vi "4Pi Interference Locator.vi"(7 "Calling VI Ref":refnum<vi>) -> ()   [LabVIEW 2021]
uses:
  <vilib>/vision/Image Controls.llb/IMAQ Image.ctl
  Hardware Configuration/Hardware Configuration Controls/Device Type.ctl
  Hardware Configuration/Hardware Configuration Controls/Device Function.ctl
  Device Library/Stages/Stages Controls/Stage Actions.ctl
  <vilib>/Utility/miscctls.llb/LVPointTypeDef.ctl
  4Pi Interference Locator Type Defs/4Pi IL Notifier Type.ctl
  4Pi Interference Locator Type Defs/4Pi IL Actions.ctl
  Device Manager/Common Device Queue/Common Device Controls/Common Device Actions.ctl
  Device Library/Cameras/Hamamatsu/Orca Flash/Orca Flash Controls/Orca Flash Actions.ctl
  Display Module/Display Module Custom Controls/ROI Descriptor.ctl
  Device Library/Stages/Stages Controls/Stage Status.ctl
  <vilib>/vision/NI_Vision_Development_Module.lvlib
panel:
  in  "Move to Cursor":bool
  in  "Halt Stage":bool
  in  "Scan Range (µm)":dbl
  out "Interference Scan":cluster{sgl[], sgl[]}(graph)
  in  "Clear Plot":bool=TRUE
  in  "Stage Settings":bool
  in  "Scan Cavity":bool
  in  "Velocity":dbl=0.001
  in  "Quit":bool
  in  "Interference Image":i32(ring) items=["Quad 01", "Quad 02", "Quad 03", "Quad 04"]
  in  "Cavity Position (µm)":dbl
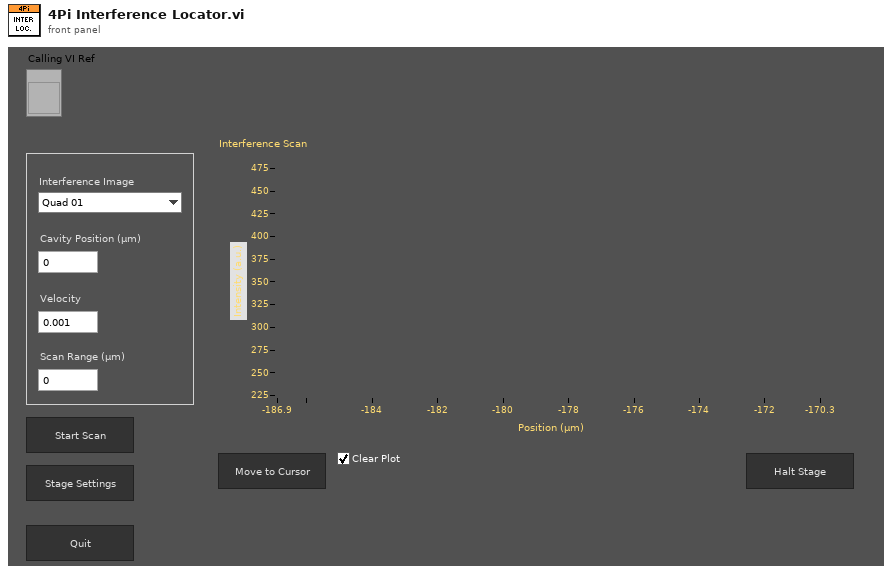
[diagram p1: front panel]
types:
  T1 = typedef "4Pi IL Actions.ctl" = enum16{"Idle", "Start Scan", "Move Stage", "Get Data", "Wait For Update", "Abort", "End Scan", "Quit"}
  T2 = typedef "4Pi IL Notifier Type.ctl" = cluster{"Actions":T1, "Image Ref":T3, "Scan Image Mask":T3}
  T3 = typedef "IMAQ Image.ctl" = refnum<image>
  T4 = enum16{"Always On", "Always Off", "Off While Running"}
  T5 = typedef "LVPointTypeDef.ctl" = cluster{"Horizontal":i16, "Vertical":i16}
  T6 = typedef "Stage Actions.ctl" = enum16{"Get Position", "SERVO OFF", "SERVO ON", "SERVO ON/OFF", "MVR", "MOVE", "HALT", "ONTARGET", "ERROR", "REFERENCE", "INIT", "VELOCITY", "STATUS", "EXIT", "HOME", "ZEROPOS", "NANOPOS", "ANALOG", "QUIT"}
  T7 = typedef "Image Type" = u32
  T8 = typedef "Device Function.ctl" = enum16{"Primary", "Secondary", "Overview", "Wide Field Drift Correction", "642 nm Excitation", "560 nm Excitation", "940 nm Excitation", "546 nm Excitation", "488 nm Excitation", "405 nm Excitation", "Objective Drift Correction", "4Pi Focus Lock", "4Pi Objective Lock", "Objective XY", "Objective Z", "Sample XY", "Sample Coarse Z", "Sample Z", "4Pi Lower", "4Pi Upper", "Em Small", "Em Large", "Ex Small", "Ex Large", "Mojo", "Adj Cavity", "Line Scanning", "Alert"}
  T9 = typedef "Device Type.ctl" = enum16{"AOTF", "Camera", "Deformable Mirror", "Laser", "Flip Mirror", "Shutter", "Stage", "Waveform", "FPGA", "Filter Wheel", "Email"}
  T10 = typedef "ROI Descriptor.ctl" = cluster{"Global Rectangle":i32[], "Contours":cluster{"Contour Type":u32, "ROI Type":u32, "Points":i32[]}[]}
  T11 = typedef "Orca Flash Actions.ctl" = enum16{"IDLE", "PREVIEW", "RECORD", "Send Trigger", "SOFT TRIGGER", "Record Settings", "SETPARAM", "GETPARAM", "SETROI", "GETROI", "PROGRESSIVE MODE", "AREA MODE", "STATUS", "QUIT"}
  T12 = typedef "Stage Status.ctl" = enum16{"Error", "Abort", "Busy", "On Target"}
  T13 = typedef "Common Device Actions.ctl" = enum16{"Specific Action", "Open Front Panel", "Close Front Panel", "Quit", "Quit All"}
  T14 = cluster{"Contour Type":u32, "ROI Type":u32, "Points":i32[]}[]
  T15 = cluster{"Contour Type":u32, "ROI Type":u32, "Points":i32[]}
  T16 = cluster{"Mean Value":sgl, "Standard Variation":sgl, "Minimal Value":sgl, "Maximal Value":sgl, "Area (calibrated)":sgl, "Area (pixels)":u32, "%":sgl, "Calibration Valid":bool}
  T17 = typedef "LVRectTypeDef.ctl" = cluster{"Left":i16, "Top":i16, "Right":i16, "Bottom":i16}
  T18 = typedef "LVBoundsTypeDef.ctl" = cluster{"Width":u32, "Height":u32}
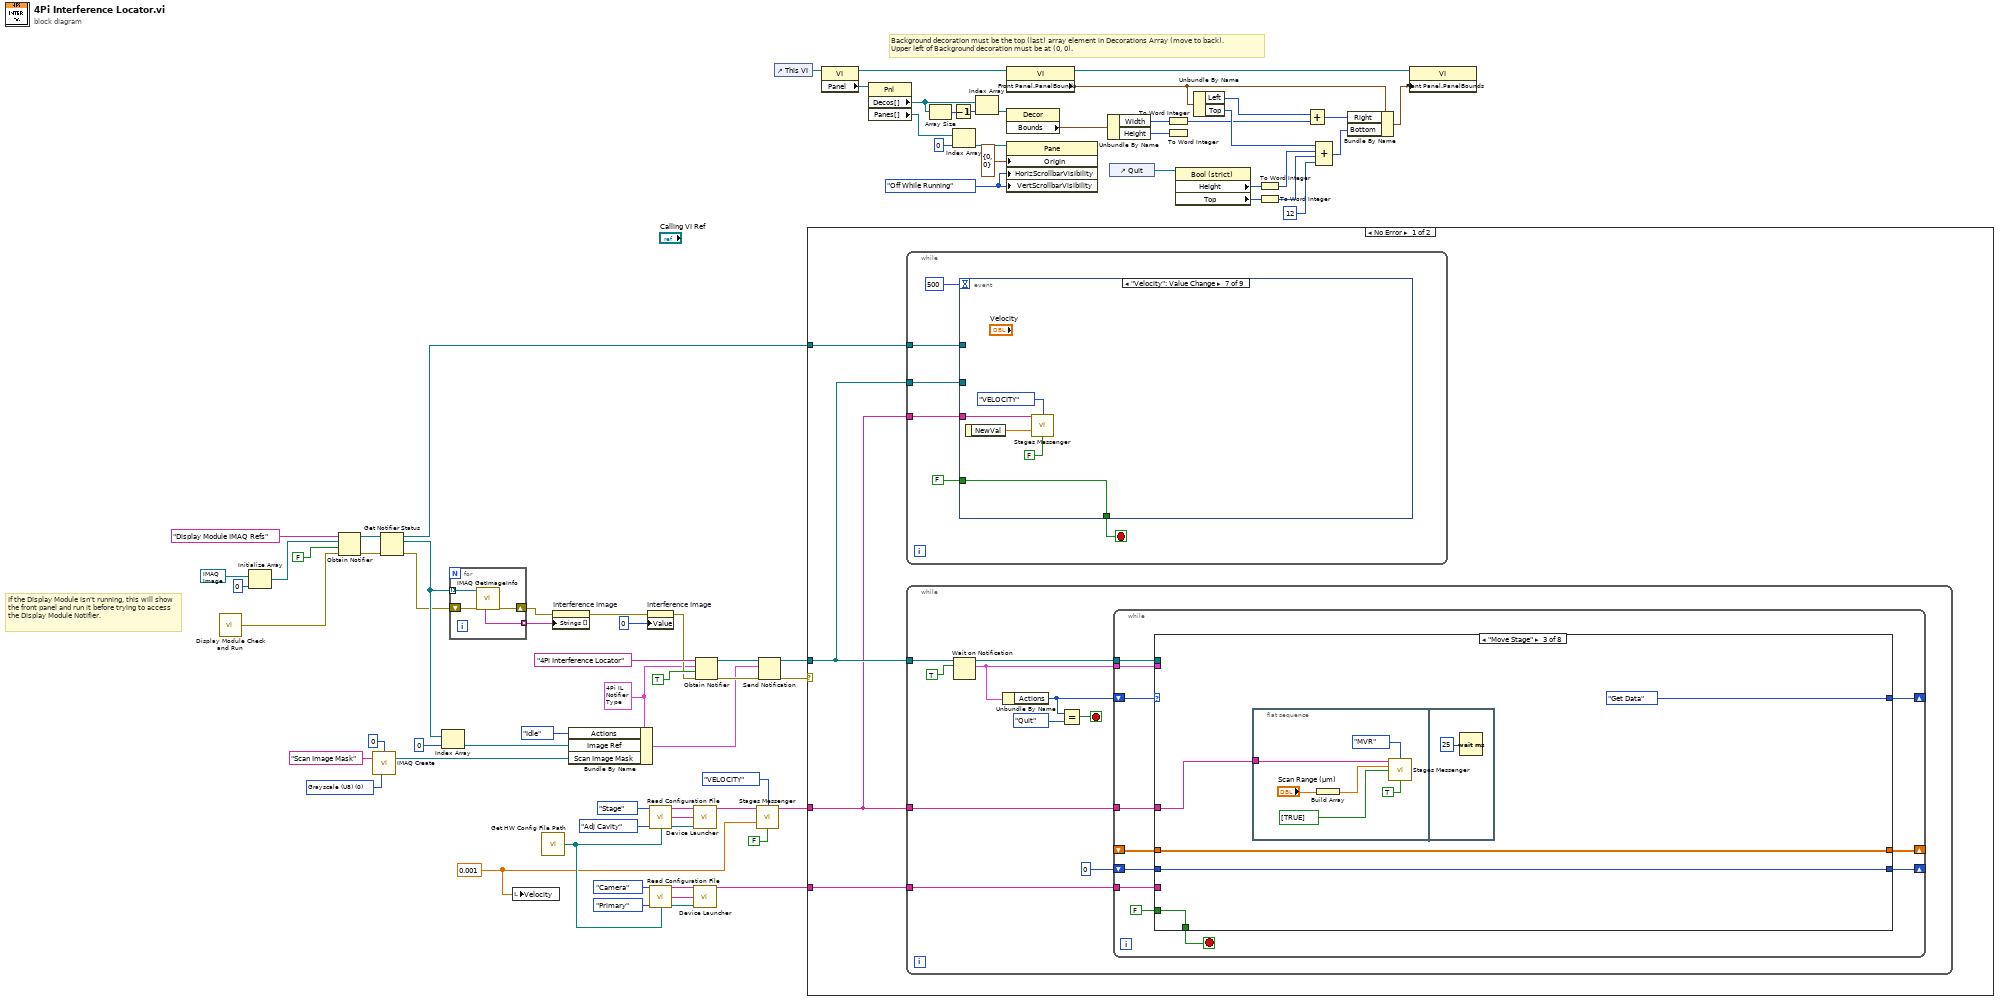
[diagram p0: block diagram]
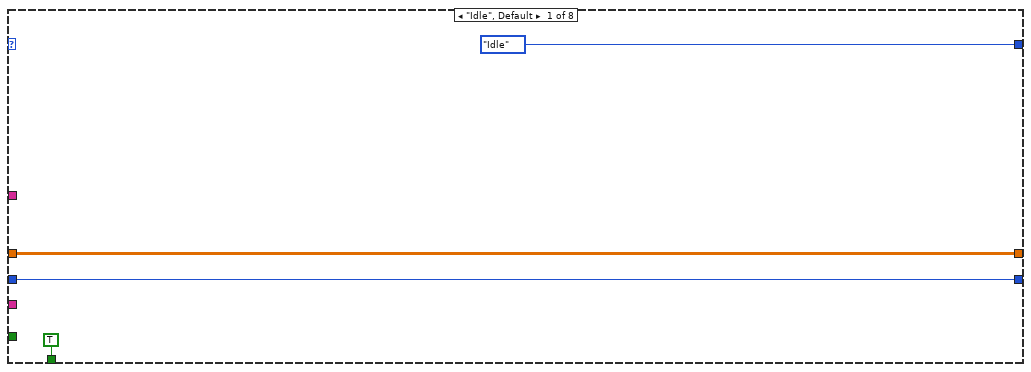
[diagram p2: hidden frame]
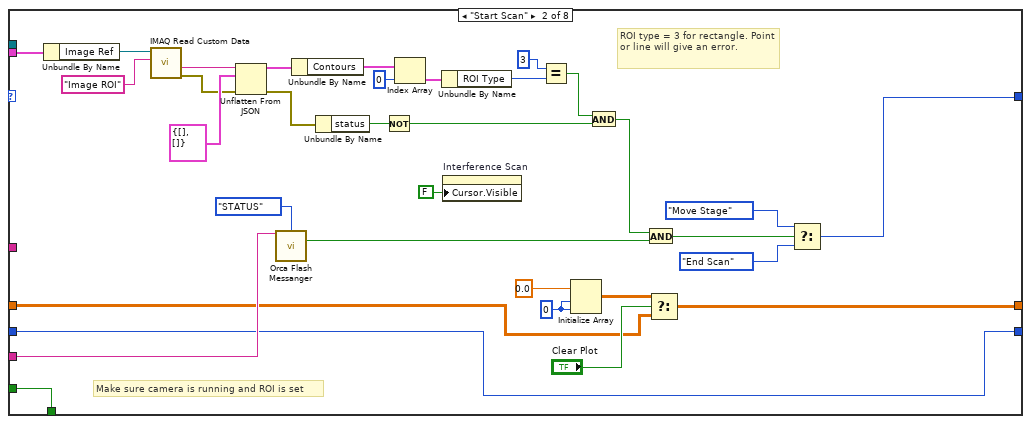
[diagram p3: hidden frame]
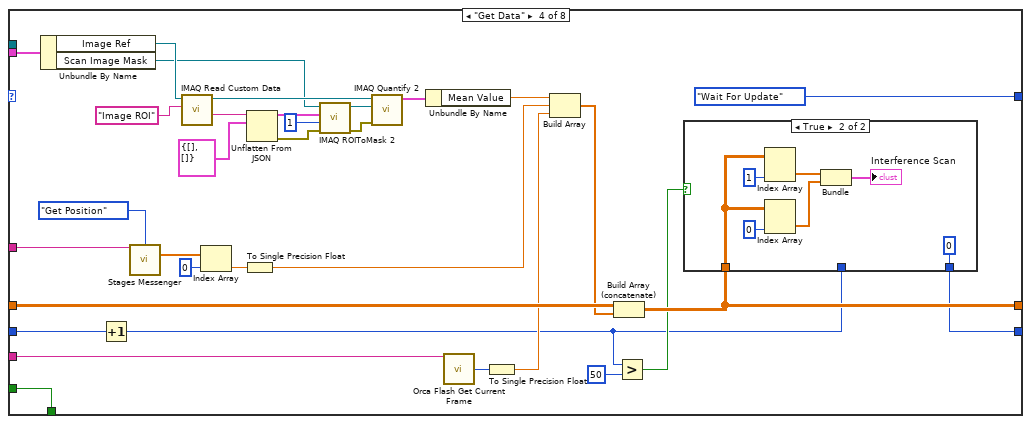
[diagram p4: hidden frame]
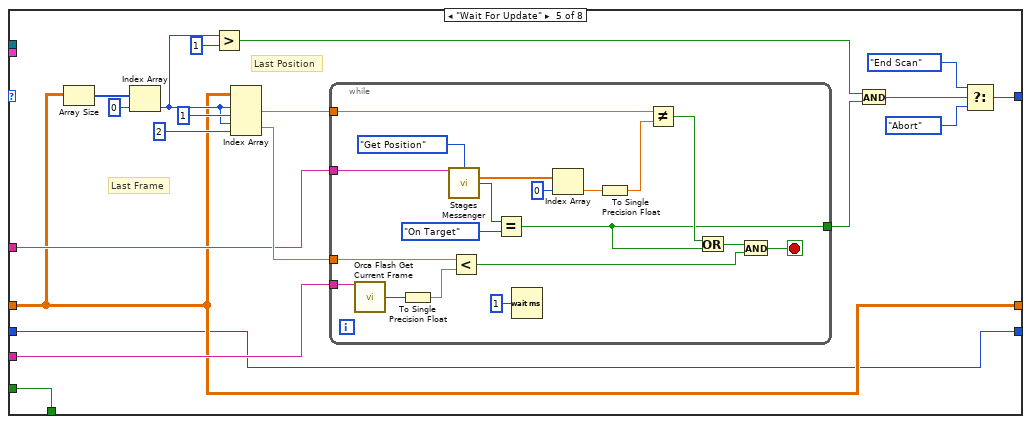
[diagram p6: hidden frame]
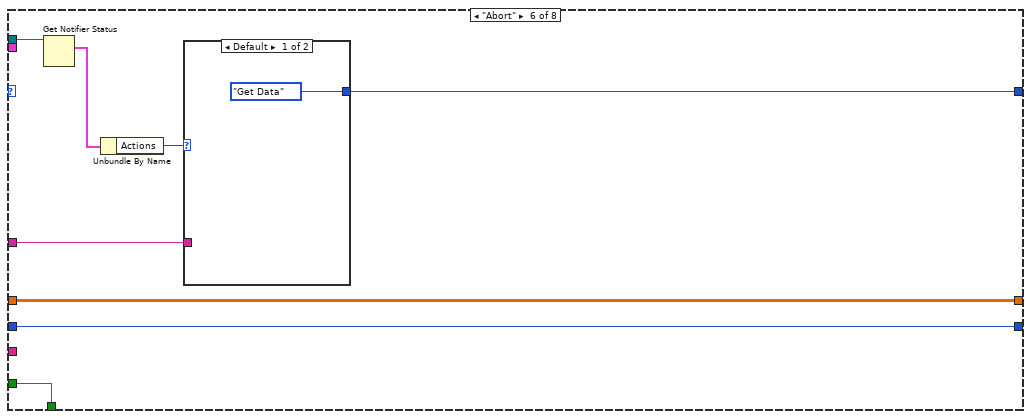
[diagram p7: hidden frame]
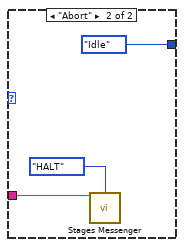
[diagram p8: hidden frame]
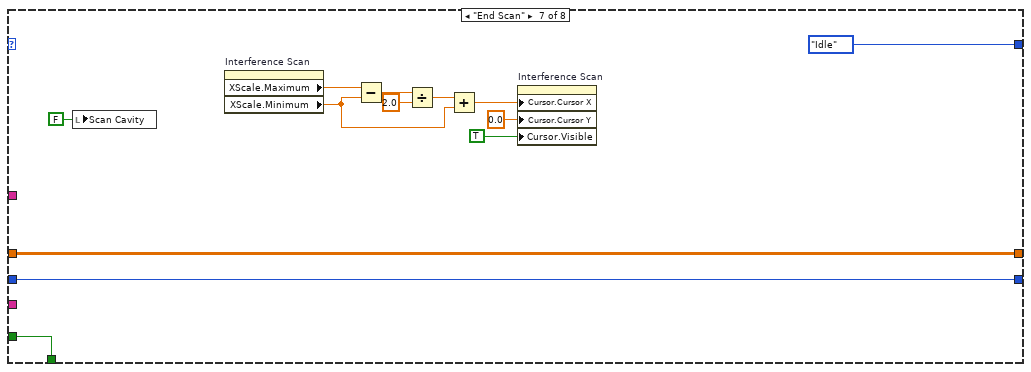
[diagram p9: hidden frame]
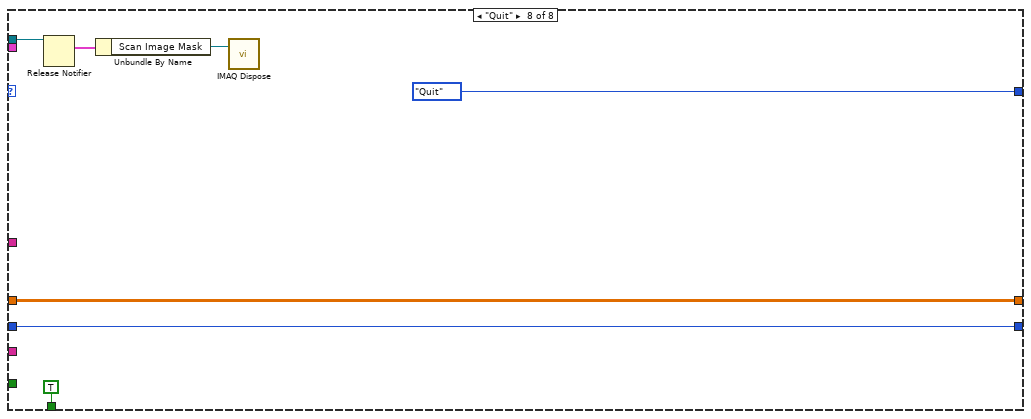
[diagram p10: hidden frame]
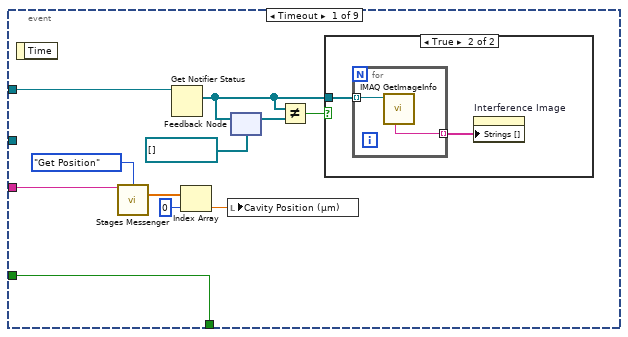
[diagram p11: hidden frame]
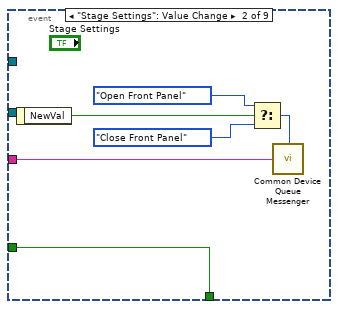
[diagram p13: hidden frame]
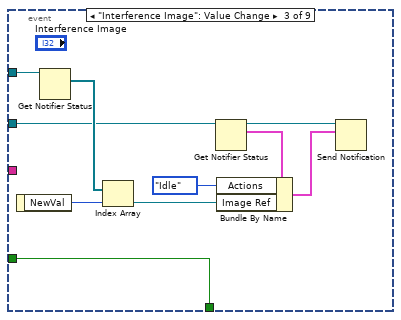
[diagram p14: hidden frame]
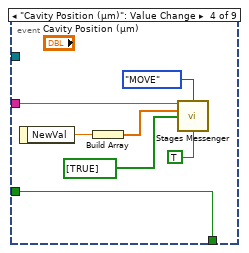
[diagram p15: hidden frame]
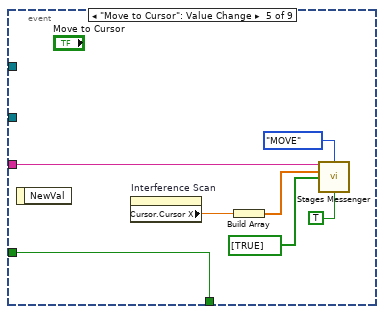
[diagram p16: hidden frame]
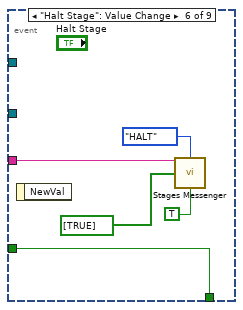
[diagram p17: hidden frame]
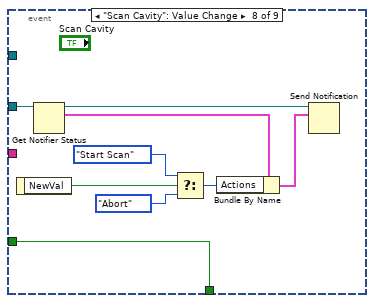
[diagram p18: hidden frame]
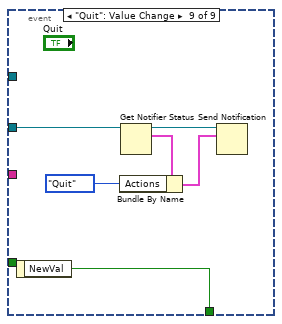
[diagram p19: hidden frame]
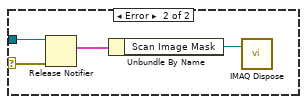
[diagram p20: hidden frame]
diagram:
  w24 = 0.001 ("element")
  w9 = T2 {"Actions"=enum."Idle", "Image Ref"=refnum, "Scan Image Mask"=refnum} ("4Pi IL Notifier Type")
  w36 = T4."Off While Running" ("Vertical Scrollbar Visibility")
  w58 = T7 0 items=["Grayscale (U8)", "Grayscale (I16)", "Grayscale (SGL)", "Complex (CSG)", "RGB (U32)", "HSL (U32)", "RGB (U64)", "Grayscale (U16)"] ("Image Type")
  # "If the Display Module isn't running, this will show the front panel and run it before trying to access the Display Module Notifier."
  # "Background decoration must be the top (last) array element in Decorations Array (move to back).\nUpper left of Background decoration must be at (0, 0)."
  n1 = call "Display Module Check and Run.vi"() -> ("Error"=w23:errorcluster)  [unwired: 15 in]
  n2 = Initialize Array(T3 refnum ("New Image"), 0 ("dimension size")) -> (w73:T3[])
  n3 = Obtain Notifier(name (unnamed)="Display Module IMAQ Refs", notification data type=w73, create if not found? (T)=FALSE, error in (no error)=w23) -> (notifier out=w72:refnum<notifier>, error out=w22:errorcluster)  [unwired: 1 out]
  n4 = call "IMAQ Create"("Border Size"=0, "Image Name"="Scan Image Mask", "Image Type"=w58) -> ("New Image"=w1:T3)  [unwired: 2 in, 1 out]
  n5 = Get Notifier Status(notifier=w72, error in (no error)=w22) -> (notifier out=w2:refnum<notifier>, current notification=w20:T3[], error out=w19:errorcluster)  [unwired: 2 out]
  n6 = Index Array(array=w20, index=0) -> (element=w7:T3)
  n7 = for {
    tunnel: w20 -> [w81] mode=indexing
    shift-right: [w79] -> w14
    shift-left: w19 -> [w80]
    tunnel: [w78] -> w18 mode=indexing
    n8 = call "IMAQ GetImageInfo"("error in (no error)"=w80, "Image"=w81) -> ("error out"=w79:errorcluster, "Image Name"=w78:string)  [unwired: 2 in, 6 out]
  }
  n9 = local write "Velocity"(w24) -> ()
  n10 = call "Get HW Config File Path.vi"() -> ("File Path"=w60:path)  [unwired: 14 in, 1 out]
  n11 = property on="Interference Image" class="Ring (strict)"(error in=w14, "Strings []"=w18) -> (error out=w21:errorcluster)  [unwired: 1 in, 1 out]
  n12 = Bundle By Name(cluster=w9, "Actions"=4Pi_IL_Actions."Idle", "Image Ref"=w7, "Scan Image Mask"=w1) -> (w6:T2)
  n13 = property on="Interference Image" class="Ring (strict)"(error in=w21, "Value"=0) -> (error out=w13:errorcluster)  [unwired: 1 in, 1 out]
  n14 = call "Read Configuration File.vi"("Device Type"=Device_Type."Stage", "Device Function"=Device_Function."Adj Cavity", "Config File Path"=w60) -> ("Unique Notifier Name"=w70:string, "Device Ports/IDs/Channels"=w68:string[], "Device Engine Path"=w69:path)  [unwired: 9 in, 1 out]
  n15 = call "Read Configuration File.vi"("Device Type"=Device_Type."Camera", "Device Function"=Device_Function."Primary", "Config File Path"=w60) -> ("Unique Notifier Name"=w61:string, "Device Ports/IDs/Channels"=w63:string[], "Device Engine Path"=w62:path)  [unwired: 9 in, 1 out]
  n16 = call "Device Launcher.vi"("Notifier Name"=w70, "Device Ports/IDs/Channels"=w68, "Device Engine Path"=w69) -> ("Notifier Name"=w54:string)  [unwired: 11 in, 1 out]
  n17 = call "Device Launcher.vi"("Notifier Name"=w61, "Device Ports/IDs/Channels"=w63, "Device Engine Path"=w62) -> ("Notifier Name"=w3:string)  [unwired: 11 in, 1 out]
  n18 = Obtain Notifier(name (unnamed)="4Pi Interference Locator", notification data type=w9, create if not found? (T)=TRUE, error in (no error)=w13) -> (notifier out=w12:refnum<notifier>, error out=w11:errorcluster)  [unwired: 1 out]
  n19 = call "Stages Messenger.vi"("Stage Notifier Name"=w54, "Actions"=Stage_Actions."VELOCITY", "Velocity"=w24, "Exit While Busy?"=FALSE) -> ("Stage Notifier Name (Dup)"=w4:string)  [unwired: 7 in, 4 out]
  n20 = Send Notification(notification=w6, notifier=w12, error in (no error)=w11) -> (notifier out=w5:refnum<notifier>, error out=w10:errorcluster)
  n21 = control-ref of="This VI"() -> (w28:refnum<vi>)
  n22 = case shown="No Error" w10 {
    selector: w10 -> [_ w345]
    tunnel: w5 -> [w85 w346]
    tunnel: w4 -> [w83 _]
    tunnel: w3 -> [w84 _]
    tunnel: w2 -> [w82 _]
    frame No Error {
      n23 = while {
        tunnel: w85 -> [w270]
        tunnel: w83 -> [w269]
        tunnel: w82 -> [w268]
        stop <- w272 stop-if-true
        n24 = event shown="[6] \"Velocity\": Value Change" {
          selector: _ -> [_ _ _ _ _ _ _ _ _]
          dyn-events: _ -> [_ _ _ _ _ _ _ _ _]
          timeout: 500 -> [_ _ _ _ _ _ _ _ _]
          tunnel: w268 -> [w284 _ w303 _ _ _ _ _ _]
          tunnel: [w280 w294 w304 w311 w318 w323 w328 w332 w343] -> w272
          tunnel: FALSE -> [w280 w294 w304 w311 w318 w323 w328 w332 _]
          tunnel: w269 -> [w279 w290 _ w308 w316 w321 w325 _ _]
          tunnel: w270 -> [_ _ w300 _ _ _ _ w336 w342]
          event Timeout {
            n25 = event-data() -> ()  [unwired: 1 in, 1 out]
            n26 = call "Stages Messenger.vi"("Stage Notifier Name"=w279, "Actions"=Stage_Actions."Get Position") -> ("Positions"=w277:dbl[])  [unwired: 9 in, 4 out]
            n27 = Get Notifier Status(notifier=w284) -> (current notification=w281:T3[])  [unwired: 1 in, 4 out]
            n28 = Index Array(array=w277, index=0) -> (element=w275:dbl)
            n29 = local write "Cavity Position (µm)"(w275) -> ()
            n30 = feedback-in #1(w281) -> ()
            n31 = feedback #1(T3[] []) -> (w283:T3[])
            n32 = Not Equal?(x=w281, y=w283) -> (x != y?=w282:bool)
            n33 = case shown="True" w282 {
              tunnel: w281 -> [_ w286]
              frame False {
              }
              frame True {
                n34 = for {
                  tunnel: w286 -> [w288] mode=indexing
                  tunnel: [w287] -> w285 mode=indexing
                  n35 = call "IMAQ GetImageInfo"("Image"=w288) -> ("Image Name"=w287:string)  [unwired: 3 in, 7 out]
                }
                n36 = property on="Interference Image" class="Ring (strict)"("Strings []"=w285) -> ()  [unwired: 2 in, 2 out]
              }
            }
          }
          event "Stage Settings": Value Change {
            n37 = event-data() -> ("NewVal"=w289:bool)  [unwired: 1 in]
            n38 = Select(t=Common_Device_Actions."Open Front Panel" ("Common Actions"), s=w289, f=Common_Device_Actions."Close Front Panel" ("Common Actions")) -> (s? t:f=w293:T13)
            n39 = call "Common Device Queue Messenger.vi"("Common Action"=w293, "Notifier Name"=w290) -> ()  [unwired: 13 in, 1 out]
          }
          event "Interference Image": Value Change {
            n40 = event-data() -> ("NewVal"=w301:i32)  [unwired: 1 in]
            n41 = Get Notifier Status(notifier=w303) -> (current notification=w302:T3[])  [unwired: 1 in, 4 out]
            n42 = Index Array(array=w302, index=w301) -> (element=w297:T3)
            n43 = Get Notifier Status(notifier=w300) -> (notifier out=w296:refnum<notifier>, current notification=w299:T2)  [unwired: 1 in, 3 out]
            n44 = Bundle By Name(cluster=w299, "Actions"=4Pi_IL_Actions."Idle", "Image Ref"=w297) -> (w295:T2)
            n45 = Send Notification(notification=w295, notifier=w296) -> ()  [unwired: 1 in, 2 out]
          }
          event "Cavity Position (µm)": Value Change {
            n46 = event-data() -> ("NewVal"=w310:dbl)  [unwired: 1 in]
            n47 = Build Array(w310) -> (w307:dbl[])
            n48 = call "Stages Messenger.vi"("Stage Notifier Name"=w308, "Actions"=Stage_Actions."MOVE", "Setpoint"=w307, "Axis"=bool[] [TRUE], "Exit While Busy?"=TRUE) -> ()  [unwired: 6 in, 5 out]
          }
          event "Move to Cursor": Value Change {
            n49 = event-data() -> ()  [unwired: 1 in, 1 out]
            n50 = property on="Interference Scan" class="XYGraph (strict)"() -> ("Cursor.Cursor X"=w312:dbl)  [unwired: 2 in, 2 out]
            n51 = Build Array(w312) -> (w315:dbl[])
            n52 = call "Stages Messenger.vi"("Stage Notifier Name"=w316, "Actions"=Stage_Actions."MOVE", "Setpoint"=w315, "Axis"=bool[] [TRUE], "Exit While Busy?"=TRUE) -> ()  [unwired: 6 in, 5 out]
          }
          event "Halt Stage": Value Change {
            n53 = event-data() -> ()  [unwired: 1 in, 1 out]
            n54 = call "Stages Messenger.vi"("Stage Notifier Name"=w321, "Actions"=Stage_Actions."HALT", "Axis"=bool[] [TRUE], "Exit While Busy?"=TRUE) -> ()  [unwired: 7 in, 5 out]
          }
          event "Velocity": Value Change {
            n55 = event-data() -> ("NewVal"=w324:dbl)  [unwired: 1 in]
            n56 = call "Stages Messenger.vi"("Stage Notifier Name"=w325, "Actions"=Stage_Actions."VELOCITY", "Velocity"=w324, "Exit While Busy?"=FALSE) -> ()  [unwired: 7 in, 5 out]
          }
          event "Scan Cavity": Value Change {
            n57 = event-data() -> ("NewVal"=w337:bool)  [unwired: 1 in]
            n58 = Get Notifier Status(notifier=w336) -> (notifier out=w329:refnum<notifier>, current notification=w335:T2)  [unwired: 1 in, 3 out]
            n59 = Select(t=4Pi_IL_Actions."Start Scan" ("Actions"), s=w337, f=4Pi_IL_Actions."Abort" ("Actions")) -> (s? t:f=w331:T1)
            n60 = Bundle By Name(cluster=w335, "Actions"=w331) -> (w330:T2)
            n61 = Send Notification(notification=w330, notifier=w329) -> ()  [unwired: 1 in, 2 out]
          }
          event "Quit": Value Change {
            n62 = event-data() -> ("NewVal"=w343:bool)  [unwired: 1 in]
            n63 = Get Notifier Status(notifier=w342) -> (notifier out=w341:refnum<notifier>, current notification=w340:T2)  [unwired: 1 in, 3 out]
            n64 = Bundle By Name(cluster=w340, "Actions"=4Pi_IL_Actions."Quit") -> (w338:T2)
            n65 = Send Notification(notification=w338, notifier=w341) -> ()  [unwired: 1 in, 2 out]
          }
        }
      }
      n66 = while {
        tunnel: w85 -> [w95]
        tunnel: w83 -> [w87]
        tunnel: w84 -> [w88]
        stop <- w91 stop-if-true
        n67 = Wait on Notification(notifier=w95, ignore previous (F)=TRUE) -> (notifier out=w89:refnum<notifier>, notification=w90:T2)  [unwired: 2 in, 2 out]
        n68 = Unbundle By Name(w90) -> ("Actions"=w92:T1)
        n69 = Equal?(x=w92, y=4Pi_IL_Actions."Quit") -> (x = y?=w91:bool)
        n70 = while {
          tunnel: w90 -> [w106]
          tunnel: w89 -> [w105]
          tunnel: w88 -> [w104]
          shift-right: [w103] -> _
          shift-left: w92 -> [w107]
          shift-right: [w100] -> _
          shift-left: _ -> [w99]
          tunnel: w87 -> [w98]
          shift-right: [w96] -> _
          shift-left: u8 0 -> [w97]
          stop <- w101 stop-if-true
          n71 = case shown="\"Move Stage\"" w107 {
            tunnel: w106 -> [_ w142 _ w188 _ _ _ _]
            tunnel: w105 -> [_ _ _ _ _ w241 _ w267]
            tunnel: w104 -> [_ w141 _ w164 w209 _ _ _]
            tunnel: [4Pi_IL_Actions."Idle" ("f") w138 4Pi_IL_Actions."Get Data" ("f") 4Pi_IL_Actions."Wait For Update" ("f") w206 w237 4Pi_IL_Actions."Idle" ("f") 4Pi_IL_Actions."Quit" ("f")] -> w103
            tunnel: FALSE -> [_ w136 w149 w189 w216 w243 w259 _]
            tunnel: [TRUE w136 w149 w189 w216 w243 w259 TRUE] -> w101
            tunnel: [w109 w131 w148 w167 w199 w242 w260 w264] -> w100
            tunnel: w99 -> [w109 w130 w148 w169 w199 w242 w260 w264]
            tunnel: w98 -> [_ _ w147 w172 w208 w238 _ _]
            tunnel: w97 -> [w108 w112 w145 w161 w198 w236 w248 w261]
            tunnel: [w108 w112 w145 w157 w198 w236 w248 w261] -> w96
            frame "Idle", Default {
            }
            frame "Start Scan" {
              w133 = 0 ("dimension size")
              # "ROI type = 3 for rectangle. Point or line will give an error."
              # "Make sure camera is running and ROI is set"
              n72 = Unbundle By Name(w142) -> ("Image Ref"=w126:T3)
              n73 = call "IMAQ Read Custom Data"("Key"="Image ROI", "Image"=w126) -> ("error out"=w125:errorcluster, "Custom Data Out"=w128:string)  [unwired: 7 in, 1 out]
              n74 = Unflatten From JSON(JSON string=w128, type and defaults=T10 {"Global Rectangle"=[], "Contours"=[]} ("Image ROI Descriptor"), error in (no error)=w125) -> (value=w119:T10, error out=w118:errorcluster)  [unwired: 4 in]
              n75 = call "Orca Flash Messanger.vi"("Notifier Name"=w141, "Camera Actions"=Orca_Flash_Actions."STATUS") -> ("Running?"=w143:bool)  [unwired: 9 in, 4 out]
              n76 = Unbundle By Name(w119) -> ("Contours"=w120:T14)
              n77 = Unbundle By Name(w118) -> ("status"=w117:bool)
              n78 = Not(x=w117) -> (.not. x?=w115:bool)
              n79 = Index Array(array=w120, index=0) -> (element=w122:T15)
              n80 = Unbundle By Name(w122) -> ("ROI Type"=w123:u32)
              n81 = property on="Interference Scan" class="XYGraph (strict)"("Cursor.Visible"=FALSE) -> ()  [unwired: 2 in, 2 out]
              n82 = Equal?(x=u32 3, y=w123) -> (x = y?=w116:bool)
              n83 = Initialize Array(sgl 0.0, w133, w133) -> (w132:sgl[][])
              n84 = And(x=w116, y=w115) -> (x .and. y?=w114:bool)
              n85 = And(x=w114, y=w143) -> (x .and. y?=w140:bool)
              n86 = Select(t=w132, s="Clear Plot", f=w130) -> (s? t:f=w131:sgl[][])
              n87 = Select(t=4Pi_IL_Actions."Move Stage" ("y"), s=w140, f=4Pi_IL_Actions."End Scan") -> (s? t:f=w138:T1)
            }
            frame "Move Stage" {
              n88 = flat-sequence {
                tunnel: w147 -> [w150]
                frame #0 {
                  n89 = Build Array("Scan Range (µm)") -> (w153:dbl[])
                  n90 = call "Stages Messenger.vi"("Stage Notifier Name"=w150, "Actions"=Stage_Actions."MVR", "Setpoint"=w153, "Axis"=bool[] [TRUE], "Exit While Busy?"=TRUE) -> ()  [unwired: 6 in, 5 out]
                }
                frame #1 {
                  n91 = Wait (ms)(milliseconds to wait=u32 25) -> ()  [unwired: 1 out]
                }
              }
            }
            frame "Get Data" {
              n92 = Unbundle By Name(w188) -> ("Image Ref"=w177:T3, "Scan Image Mask"=w176:T3)
              n93 = Increment(x=w161) -> (x+1=w158:u8)
              n94 = call "Stages Messenger.vi"("Stage Notifier Name"=w172, "Actions"=Stage_Actions."Get Position") -> ("Positions"=w175:dbl[])  [unwired: 9 in, 4 out]
              n95 = call "IMAQ Read Custom Data"("Key"="Image ROI", "Image"=w177) -> ("Custom Data Out"=w186:string, "Image (duplicate)"=w178:T3)  [unwired: 7 in, 1 out]
              n96 = Index Array(array=w175, index=0) -> (element=w171:dbl)
              n97 = To Single Precision Float(number=w171) -> (single precision float=w170:sgl)
              n98 = Unflatten From JSON(JSON string=w186, type and defaults=T10 {"Global Rectangle"=[], "Contours"=[]} ("Image ROI Descriptor")) -> (value=w184:T10, error out=w180:errorcluster)  [unwired: 5 in]
              n99 = call "IMAQ ROIToMask 2"("error in (no error)"=w180, "Filling Value (255)"=1, "ROI Descriptor"=w184, "Image"=w176) -> ("error out"=w181:errorcluster, "Image Out"=w182:T3)  [unwired: 5 in, 1 out]
              n100 = call "IMAQ Quantify 2"("error in (no error)"=w181, "Image Mask"=w182, "Image"=w178) -> ("Global Report"=w179:T16)  [unwired: 6 in, 2 out]
              n101 = Unbundle By Name(w179) -> ("Mean Value"=w165:sgl)
              n102 = call "Orca Flash Get Current Frame.vi"("Camera Notifier Name"=w164) -> ("Current Frame"=w163:u32)  [unwired: 13 in, 1 out]
              n103 = To Single Precision Float(number=w163) -> (single precision float=w162:sgl)
              n104 = Build Array(w165, w170, w162) -> (w168:sgl[])
              n105 = Build Array (concatenate)(w169, w168) -> (w167:sgl[][])
              n106 = Greater?(x=w158, y=u8 50) -> (0:w159:bool)
              n107 = case shown="True" w159 {
                tunnel: w167 -> [_ w193]
                tunnel: w158 -> [w190 _]
                tunnel: [w190 u8 0] -> w157
                frame False {
                }
                frame True {
                  n108 = Index Array(array=w193, index (col)=1 ("disabled index (col)")) -> (element=w195:sgl[])  [unwired: 1 in]
                  n109 = Index Array(array=w193, index (col)=0 ("disabled index (col)")) -> (element=w194:sgl[])  [unwired: 1 in]
                  n110 = Bundle(w195, w194) -> (→"Interference Scan":cluster{sgl[], sgl[]})  [unwired: 1 in]
                }
              }
            }
            frame "Wait For Update" {
              # "Last Frame"
              # "Last Position"
              n111 = Array Size(array=w199) -> (size(s)=w215:i32[])
              n112 = Index Array(array=w215, index=0) -> (element=w204:i32)
              n113 = Greater?(x=w204, y=1) -> (0:w201:bool)
              n114 = Index Array(array=w199, index (row) #1=w204, index (col) #1=1 ("disabled index (col)"), index (row) #2=w204, index (col) #2=2 ("disabled index (col)")) -> (element #1=w211:sgl, element #2=w210:sgl)
              n115 = while {
                tunnel: w210 -> [w233]
                tunnel: w209 -> [w232]
                tunnel: w208 -> [w228]
                tunnel: w211 -> [w227]
                tunnel: [w217] -> w202
                stop <- w219 stop-if-true
                n116 = call "Orca Flash Get Current Frame.vi"("Camera Notifier Name"=w232) -> ("Current Frame"=w235:u32)  [unwired: 13 in, 1 out]
                n117 = To Single Precision Float(number=w235) -> (single precision float=w234:sgl)
                n118 = call "Stages Messenger.vi"("Stage Notifier Name"=w228, "Actions"=Stage_Actions."Get Position") -> ("Positions"=w226:dbl[], "Status"=w230:T12)  [unwired: 9 in, 3 out]
                n119 = Less?(x=w233, y=w234) -> (x < y?=w220:bool)
                n120 = Equal?(x=w230, y=Stage_Status."On Target") -> (x = y?=w217:bool)
                n121 = Wait (ms)(milliseconds to wait=u32 1) -> ()  [unwired: 1 out]
                n122 = Index Array(array=w226, index=0) -> (element=w224:dbl)
                n123 = To Single Precision Float(number=w224) -> (single precision float=w223:sgl)
                n124 = Not Equal?(x=w227, y=w223) -> (x != y?=w222:bool)
                n125 = Or(x=w222, y=w217) -> (x .or. y?=w221:bool)
                n126 = And(x=w221, y=w220) -> (x .and. y?=w219:bool)
              }
              n127 = And(x=w201, y=w202) -> (x .and. y?=w200:bool)
              n128 = Select(t=4Pi_IL_Actions."End Scan" ("y"), s=w200, f=4Pi_IL_Actions."Abort" ("y")) -> (s? t:f=w206:T1)
            }
            frame "Abort" {
              n129 = Get Notifier Status(notifier=w241) -> (current notification=w240:T2)  [unwired: 1 in, 4 out]
              n130 = Unbundle By Name(w240) -> ("Actions"=w239:T1)
              n131 = case shown="Default" w239 {
                tunnel: w238 -> [_ w247]
                tunnel: [4Pi_IL_Actions."Get Data" ("f") 4Pi_IL_Actions."Idle" ("f")] -> w237
                frame Default {
                }
                frame "Abort" {
                  n132 = call "Stages Messenger.vi"("Stage Notifier Name"=w247, "Actions"=Stage_Actions."HALT") -> ()  [unwired: 9 in, 5 out]
                }
              }
            }
            frame "End Scan" {
              n133 = local write "Scan Cavity"(FALSE ("Scan Cavity")) -> ()
              n134 = property on="Interference Scan" class="XYGraph (strict)"() -> ("XScale.Maximum"=w256:dbl, "XScale.Minimum"=w249:dbl)  [unwired: 2 in, 2 out]
              n135 = Subtract(x=w256, y=w249) -> (x-y=w253:dbl)
              n136 = Divide(x=w253, y=2.0) -> (x/y=w251:dbl)
              n137 = Add(x=w251, y=w249) -> (x+y=w250:dbl)
              n138 = property on="Interference Scan" class="XYGraph (strict)"("Cursor.Cursor X"=w250, "Cursor.Cursor Y"=0.0 ("Cursor.Cursor Position:Cursor Y"), "Cursor.Visible"=TRUE) -> ()  [unwired: 2 in, 2 out]
            }
            frame "Quit" {
              n139 = Release Notifier(notifier=w267) -> (last notification=w262:T2)  [unwired: 2 in, 2 out]
              n140 = Unbundle By Name(w262) -> ("Scan Image Mask"=w263:T3)
              n141 = call "IMAQ Dispose"("Image"=w263) -> ()  [unwired: 5 in, 1 out]
            }
          }
        }
      }
    }
    frame Error {
      n142 = Release Notifier(notifier=w346, error in (no error)=w345) -> (last notification=w344:T2)  [unwired: 1 in, 2 out]
      n143 = Unbundle By Name(w344) -> ("Scan Image Mask"=w347:T3)
      n144 = call "IMAQ Dispose"("Image"=w347) -> ()  [unwired: 5 in, 1 out]
    }
  }
  n145 = property class="VI"(reference=w28) -> (reference out=w37:refnum<vi>, "Panel"=w29:refnum<vi>)  [unwired: 1 in, 1 out]
  n146 = property class="Pnl"(reference=w29) -> ("Decos[]"=w27:refnum<vi>[], "Panes[]"=w33:refnum<vi>[])  [unwired: 1 in, 2 out]
  n147 = Array Size(array=w27) -> (size(s)=w25:i32)
  n148 = Decrement(x=w25) -> (x-1=w26:i32)
  n149 = Index Array(array=w33, index=0) -> (element=w32:refnum<vi>)
  n150 = Index Array(array=w27, index=w26) -> (element=w35:refnum<vi>)
  n151 = property class="VI"(reference=w37) -> (reference out=w39:refnum<vi>, "Front Panel.PanelBounds"=w40:T17)  [unwired: 1 in, 1 out]
  n152 = property class="Decor"(reference=w35) -> ("Bounds"=w38:T18)  [unwired: 1 in, 2 out]
  n153 = property class="Pane"(reference=w32, "Origin"=T5 {"Horizontal"=0, "Vertical"=0}, "HorizScrollbarVisibility"=w36, "VertScrollbarVisibility"=w36) -> ()  [unwired: 1 in, 2 out]
  n154 = Unbundle By Name(w38) -> ("Width"=w43:u32, "Height"=w46:u32)
  n155 = control-ref of="Quit"() -> (w30:refnum<vi>)
  n156 = To Word Integer(number=w43) -> (16bit integer=w45:i16)
  n157 = To Word Integer(number=w46) -> ()  [unwired: 1 out]
  n158 = property class="Bool (strict)"(reference=w30) -> ("Height"=w48:u32, "Top"=w49:i32)  [unwired: 1 in, 2 out]
  n159 = Unbundle By Name(w40) -> ("Left"=w42:i16, "Top"=w53:i16)
  n160 = To Word Integer(number=w48) -> (16bit integer=w51:i16)
  n161 = To Word Integer(number=w49) -> (16bit integer=w52:i16)
  n162 = Add(x=w42, y=w45) -> (x+y=w44:i16)
  n163 = Compound Arithmetic op=ADD(w53, w51, w52, i16 12 ("y")) -> (w47:i16)
  n164 = Bundle By Name(cluster=w40, "Right"=w44, "Bottom"=w47) -> (w41:T17)
  n165 = property class="VI"(reference=w39, "Front Panel.PanelBounds"=w41) -> ()  [unwired: 1 in, 2 out]
